vi "UNO Q AnalogRead.vi"(8 "error in (no error)":errorcluster, 10 "Analog pin":T1, 11 "UNO Q Session in":T2={"HTTP client"=refnum, "Base URL"="", "Connected"=TRUE}) -> (0 "error out":errorcluster, 2 "values":i32[](array[numeric]), 3 "UNO Q Session out":T2={"HTTP client"=refnum, "Base URL"="", "Connected"=TRUE}, 4 "status":i32, 6 "error":string)   [LabVIEW 2021]
uses:
  UNO Q Session.ctl
  <vilib>/httpClient/ClientHandle.ctl
  Apin typedef.ctl
  ERR typedef.ctl
  <vilib>/httpClient/POSTBuffer.vi
  <vilib>/httpClient/LabVIEWHTTPClient.lvlib
panel:
  out "headers":string
  out "body":string
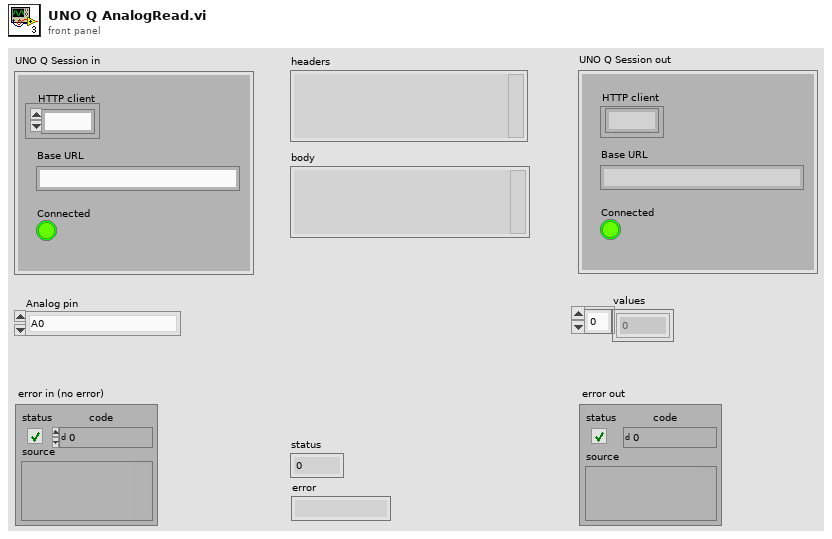
[diagram p1: front panel]
types:
  T1 = typedef "Apin typedef.ctl" = enum16{"A0", "A1", "A2", "A3", "A4", "A5"}
  T2 = typedef "UNO Q Session.ctl" = cluster{"HTTP client":T3, "Base URL":string, "Connected":bool}
  T3 = typedef "LabVIEWHTTPClient.lvlib/ClientHandle.ctl" = refnum<k1>
  T4 = typedef "ERR typedef.ctl" = enum16{"STATUS OK", "STATUS INVALID ARGUMENT", "STATUS NOT IMPLEMENTED", "STATUS RUNTIME ERROR"}
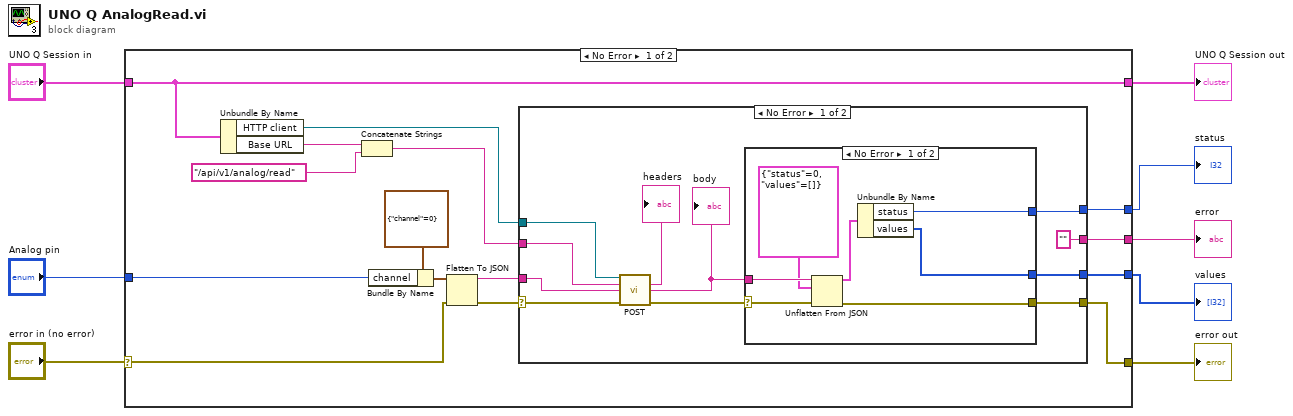
[diagram p0: block diagram]
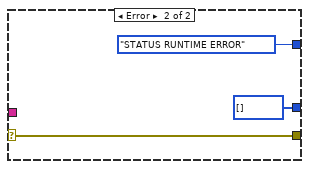
[diagram p2: hidden frame]
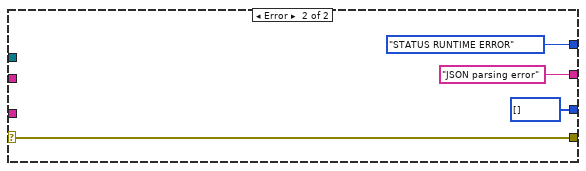
[diagram p3: hidden frame]
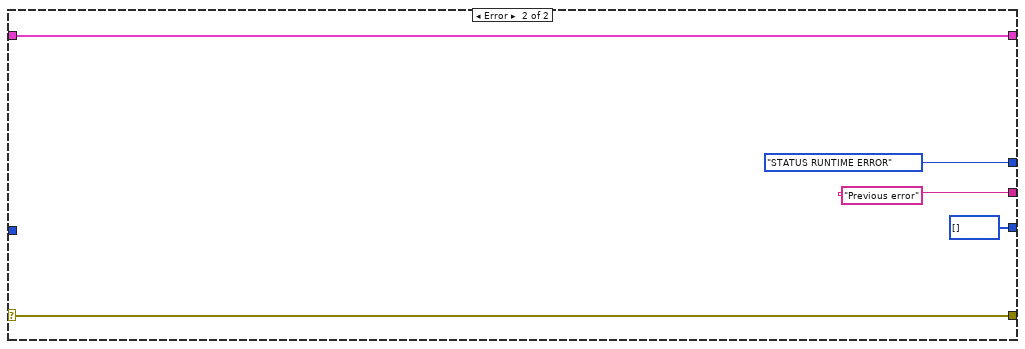
[diagram p4: hidden frame]
diagram:
  n1 = case shown="No Error" "error in (no error)" {
    selector: "error in (no error)" -> [w17 w53]
    tunnel: [w15 w53] -> w7
    tunnel: "UNO Q Session in" -> [w21 w52]
    tunnel: [w21 w52] -> w5
    tunnel: [w14 ERR_typedef."STATUS RUNTIME ERROR" ("Error code")] -> w4
    tunnel: [w13 "Previous error" ("error")] -> w3
    tunnel: "Analog pin" -> [w10 _]
    tunnel: [w9 i32[] [] ("values")] -> w1
    frame No Error {
      n2 = Unbundle By Name(w21) -> ("HTTP client"=w20:T3, "Base URL"=w23:string)
      n3 = Concatenate Strings(w23, "/api/v1/analog/read" ("string")) -> (w19:string)
      n4 = Bundle By Name(cluster=cluster{"channel":i32} {"channel"=0}, "channel"=w10) -> (w12:cluster{"channel":i32})
      n5 = Flatten To JSON(anything=w12, error in (no error)=w17) -> (JSON string=w18:string, 11:w16:errorcluster)  [unwired: 1 in]
      n6 = case shown="No Error" w16 {
        selector: w16 -> [w30 w48]
        tunnel: w20 -> [w34 _]
        tunnel: w19 -> [w33 _]
        tunnel: w18 -> [w32 _]
        tunnel: [w27 w48] -> w15
        tunnel: [w25 ERR_typedef."STATUS RUNTIME ERROR" ("Error code")] -> w14
        tunnel: ["" ("error") "JSON parsing error" ("error")] -> w13
        tunnel: [w24 i32[] [] ("values")] -> w9
        frame No Error {
          n7 = call-poly <vilib>:"POST.vi"("client handle"=w34, "url"=w33, "buffer"=w32, "error in (no error)"=w30) -> ("headers"=→"headers":string, "body"=w26:string, "error out"=w28:errorcluster)  [unwired: 8 in, 1 out]
          "body" <- w26
          n8 = case shown="No Error" w28 {
            selector: w28 -> [w41 w44]
            tunnel: [w38 w44] -> w27
            tunnel: w26 -> [w40 _]
            tunnel: [w36 ERR_typedef."STATUS RUNTIME ERROR" ("Error code")] -> w25
            tunnel: [w35 i32[] [] ("values")] -> w24
            frame No Error {
              n9 = Unflatten From JSON(JSON string=w40, type and defaults=cluster{"status":i32, "values":i32[]} {"status"=0, "values"=[]}, error in (no error)=w41) -> (value=w37:cluster{"status":i32, "values":i32[]}, error out=w38:errorcluster)  [unwired: 4 in]
              n10 = Unbundle By Name(w37) -> ("status"=w36:i32, "values"=w35:i32[])
            }
            frame Error {
            }
          }
        }
        frame Error {
        }
      }
    }
    frame Error {
    }
  }
  "error out" <- w7
  "UNO Q Session out" <- w5
  "status" <- w4
  "error" <- w3
  "values" <- w1
